vi "OnCommand(SingleObject).vi"(10 "Command ID":string, 11 "Object":T1) -> ()   [LabVIEW 2017]
uses:
  <resource>/Framework/Providers/API/ItemRef.ctl
  user.lib/_NEVSTOP/Communicable State Machine(CSM)/_xnode/csm_tool/_xnode_csm_tool_support/CSM DebugTool Dialog.lvlib
  user.lib/_NEVSTOP/Communicable State Machine(CSM)/_Shared/CSM Shared.lvlib
panel:
  # "PROJFILE_TRIGGER_BUILDSYSTEM\nPROJFILE_TRIGGER_TESTSYSTEM"
  # "VFOLDER_TRIGGER_BUILDSYSTEM\nVFOLDER_TRIGGER_TESTSYSTEM"
  # "ToolProviders_SCANTOOLS\nToolProviders_xxxxx"
  # "PINMAPFILE_xxxxxx"
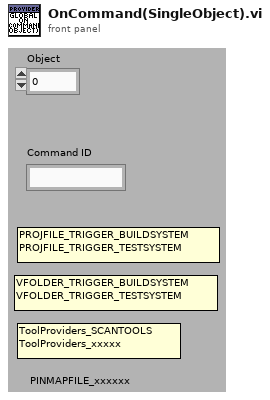
[diagram p1: front panel]
types:
  T1 = typedef "ItemRef.ctl" = u64
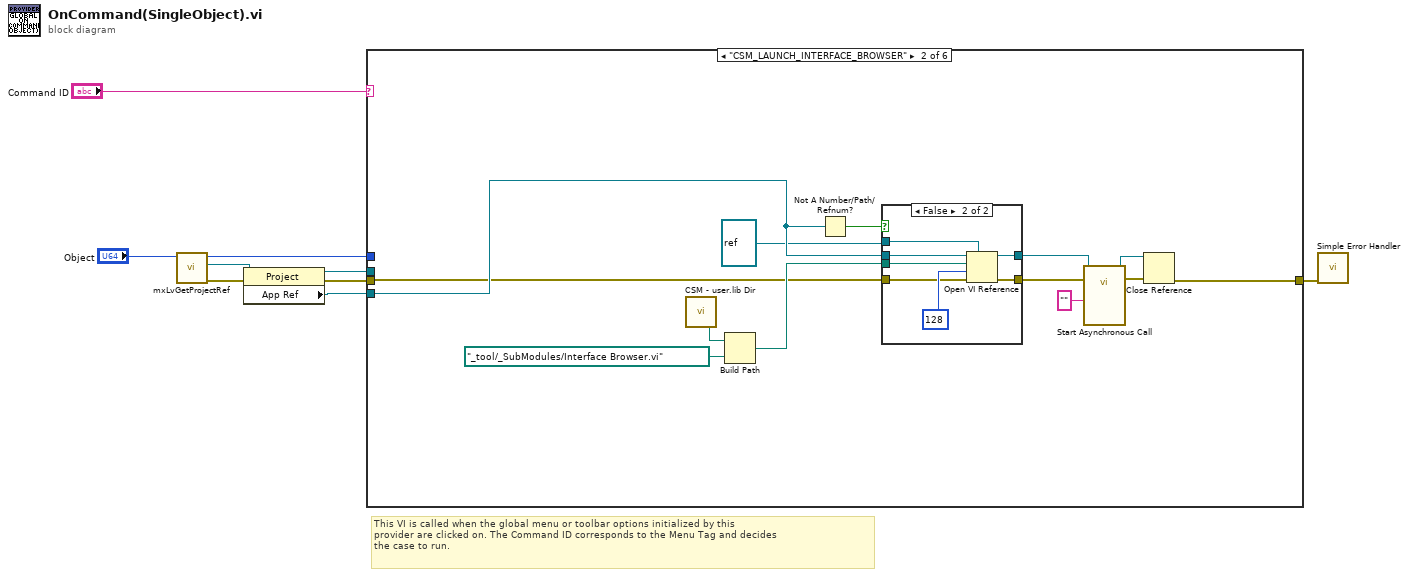
[diagram p0: block diagram]
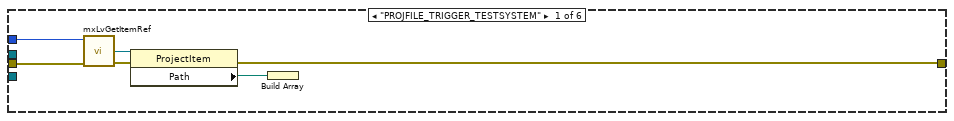
[diagram p2: hidden frame]
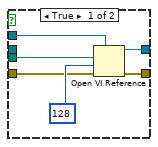
[diagram p3: hidden frame]
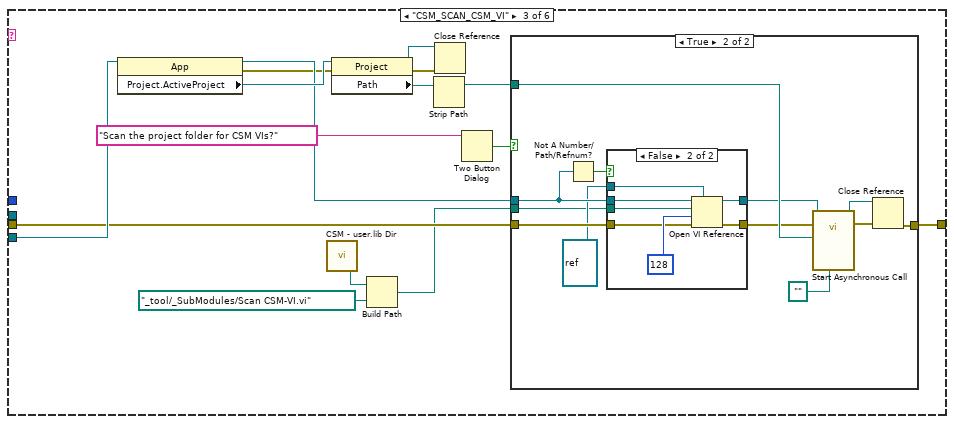
[diagram p4: hidden frame]
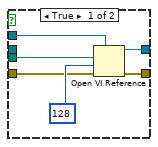
[diagram p6: hidden frame]
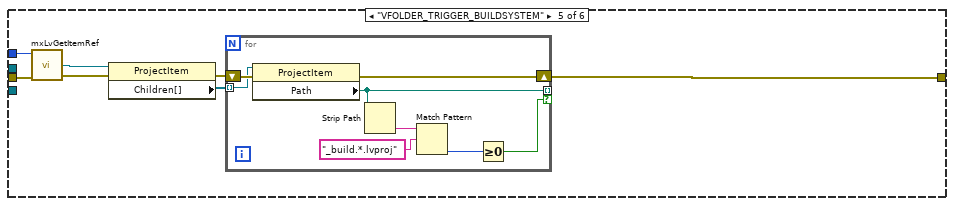
[diagram p8: hidden frame]
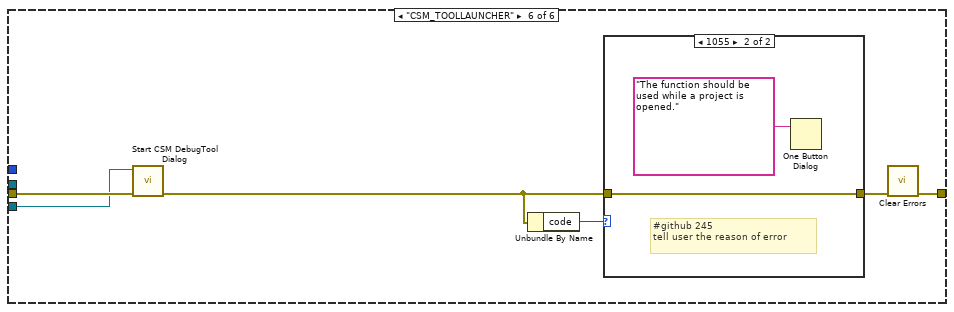
[diagram p9: hidden frame]
diagram:
  # "This VI is called when the global menu or toolbar options initialized by this \nprovider are clicked on. The Command ID corresponds to the Menu Tag and decides\nthe case to run."
  n1 = call <resource>:"mxLvGetProjectRef.vi"("Item"="Object") -> ("error out"=w8:errorcluster, "Project Refnum"=w7:refnum<vi>, "Item"=w5:T1)  [unwired: 8 in]
  n2 = property class="Project"(reference=w7, error in=w8) -> (reference out=w3:refnum<vi>, error out=w4:errorcluster, "App Ref"=w2:refnum<vi>)
  n3 = case shown="\"CSM_LAUNCH_INTERFACE_BROWSER\"" "Command ID" {
    tunnel: [w11 w21 w47 w83 w86 w99] -> w1
    tunnel: w5 -> [w13 _ _ _ w90 _]
    tunnel: w4 -> [w12 w18 w49 w83 w89 w103]
    tunnel: w2 -> [_ w22 w50 _ _ w102]
    tunnel: w3 -> [_ _ _ _ _ _]
    frame "PROJFILE_TRIGGER_TESTSYSTEM" {
      n4 = call <resource>:"mxLvGetItemRef.vi"("Item"=w13, "error in"=w12) -> ("Item Refnum"=w15:refnum<vi>, "error out"=w14:errorcluster)  [unwired: 1 out]
      n5 = property class="ProjectItem"(reference=w15, error in=w14) -> (error out=w11:errorcluster, "Path"=w10:path)  [unwired: 1 out]
      n6 = Build Array(w10) -> ()  [unwired: 1 out]
    }
    frame "CSM_LAUNCH_INTERFACE_BROWSER" {
      n7 = call "CSM - user.lib Dir.vi"() -> ("csm_user.lib_dir"=w20:path)  [unwired: 2 in, 1 out]
      n8 = Build Path(base path=w20, name or relative path=path "_tool/_SubModules/Interface Browser.vi" ("execute path")) -> (appended path=w19:path)
      n9 = Not A Number/Path/Refnum?(number/path/refnum=w22) -> (NaN/Path/Refnum?=w23:bool)
      n10 = case shown="False" w23 {
        tunnel: refnum<vi> refnum -> [w33 w40]
        tunnel: [w32 w39] -> w25
        tunnel: w18 -> [w31 w38]
        tunnel: w19 -> [w30 w37]
        tunnel: [w29 w36] -> w24
        tunnel: w22 -> [_ w35]
        frame True {
          n11 = Open VI Reference(type specifier VI Refnum (for type only)=w33, vi path=w30, options=128, error in (no error)=w31) -> (vi reference=w32:refnum<vi>, error out=w29:errorcluster)  [unwired: 2 in]
        }
        frame False {
          n12 = Open VI Reference(type specifier VI Refnum (for type only)=w40, application reference (local)=w35, vi path=w37, options=128, error in (no error)=w38) -> (vi reference=w39:refnum<vi>, error out=w36:errorcluster)  [unwired: 1 in]
        }
      }
      n13 = call-by-ref "Start Asynchronous Call"(reference=w25, error in=w24, "Init State(\"Macro: Initialize\")"="" ("Init State(\"Macro: Initialize\")")) -> (reference out=w27:refnum<vi>, error out=w26:errorcluster)  [unwired: 11 in]
      n14 = Close Reference(reference=w27, error in (no error)=w26) -> (error out=w21:errorcluster)
    }
    frame "CSM_SCAN_CSM_VI" {
      n15 = property class="App"(reference=w50) -> (reference out=w51:refnum<vi>, error out=w45:errorcluster, "Project.ActiveProject"=w52:refnum<vi>)  [unwired: 1 in]
      n16 = call "CSM - user.lib Dir.vi"() -> ("csm_user.lib_dir"=w55:path)  [unwired: 2 in, 1 out]
      n17 = property class="Project"(reference=w52, error in=w45) -> (reference out=w44:refnum<vi>, error out=w46:errorcluster, "Path"=w53:path)
      n18 = Build Path(base path=w55, name or relative path=path "_tool/_SubModules/Scan CSM-VI.vi" ("execute path")) -> (appended path=w48:path)
      n19 = Strip Path(path=w53) -> (stripped path=w54:path)  [unwired: 1 out]
      n20 = Close Reference(reference=w44, error in (no error)=w46) -> ()  [unwired: 1 out]
      n21 = Two Button Dialog(message="Scan the project folder for CSM VIs?") -> (T button?=w43:bool)  [unwired: 2 in]
      n22 = case shown="True" w43 {
        tunnel: w54 -> [_ w69]
        tunnel: w51 -> [_ w68]
        tunnel: w49 -> [w57 w61]
        tunnel: w48 -> [_ w59]
        tunnel: [w57 w58] -> w47
        frame False {
        }
        frame True {
          n23 = Not A Number/Path/Refnum?(number/path/refnum=w68) -> (NaN/Path/Refnum?=w67:bool)
          n24 = case shown="False" w67 {
            tunnel: refnum<vi> refnum -> [w74 w81]
            tunnel: [w73 w80] -> w65
            tunnel: w61 -> [w72 w79]
            tunnel: w59 -> [w71 w78]
            tunnel: [w70 w77] -> w66
            tunnel: w68 -> [_ w76]
            frame True {
              n25 = Open VI Reference(type specifier VI Refnum (for type only)=w74, vi path=w71, options=128, error in (no error)=w72) -> (vi reference=w73:refnum<vi>, error out=w70:errorcluster)  [unwired: 2 in]
            }
            frame False {
              n26 = Open VI Reference(type specifier VI Refnum (for type only)=w81, application reference (local)=w76, vi path=w78, options=128, error in (no error)=w79) -> (vi reference=w80:refnum<vi>, error out=w77:errorcluster)  [unwired: 1 in]
            }
          }
          n27 = call-by-ref "Start Asynchronous Call"(reference=w65, error in=w66, "Config Path"=path "", "root"=w69) -> (reference out=w63:refnum<vi>, error out=w64:errorcluster)  [unwired: 9 in, 1 out]
          n28 = Close Reference(reference=w63, error in (no error)=w64) -> (error out=w58:errorcluster)
        }
      }
    }
    frame Default {
    }
    frame "VFOLDER_TRIGGER_BUILDSYSTEM" {
      n29 = call <resource>:"mxLvGetItemRef.vi"("Item"=w90, "error in"=w89) -> ("Item Refnum"=w84:refnum<vi>, "error out"=w85:errorcluster)  [unwired: 1 out]
      n30 = property class="ProjectItem"(reference=w84, error in=w85) -> (error out=w87:errorcluster, "Children[]"=w88:refnum<vi>[])  [unwired: 1 out]
      n31 = for {
        shift-right: [w97] -> w86
        shift-left: w87 -> [w98]
        tunnel: w88 -> [w96] mode=indexing
        tunnel: [w95] -> _ mode=indexing if=w91
        n32 = property class="ProjectItem"(reference=w96, error in=w98) -> (error out=w97:errorcluster, "Path"=w95:path)  [unwired: 1 out]
        n33 = Strip Path(path=w95) -> (name=w92:string)  [unwired: 1 out]
        n34 = Match Pattern(string=w92, regular expression="_build.*.lvproj") -> (offset past match=w94:i32)  [unwired: 1 in, 3 out]
        n35 = Greater Or Equal To 0?(x=w94) -> (x >= 0?=w91:bool)
      }
    }
    frame "CSM_TOOLLAUNCHER" {
      n36 = call "Start CSM DebugTool Dialog.vi"("error in (no error)"=w103, "Application In"=w102) -> ("error out"=w101:errorcluster)  [unwired: 9 in]
      n37 = Unbundle By Name(w101) -> ("code"=w100:i32)
      n38 = case shown="1055" w100 {
        tunnel: [w105 w107] -> w104
        tunnel: w101 -> [w105 w107]
        frame 0, Default {
        }
        frame 1055 {
          # "#github 245\ntell user the reason of error"
          n39 = One Button Dialog(message="The function should be used while a project is opened.") -> ()  [unwired: 1 in, 1 out]
        }
      }
      n40 = call <vilib>:"Clear Errors.vi"("error in (no error)"=w104) -> ("error out"=w99:errorcluster)  [unwired: 5 in, 1 out]
    }
  }
  n41 = call <vilib>:"Simple Error Handler.vi"("error in (no error)"=w1) -> ()  [unwired: 4 in, 5 out]
